vi "OwnFile20261012_Native_GetWireBroken.vi"() -> ()   [LabVIEW 2024]
panel:
  out "error out":errorcluster caption="错误输出"
  out "is_broken":bool
  in  "wire_id":u32
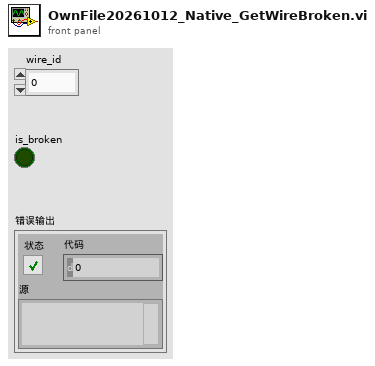
[diagram p1: front panel]
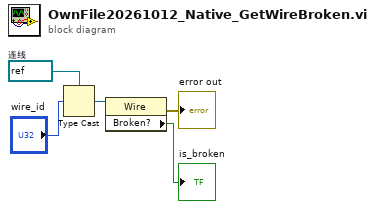
[diagram p0: block diagram]
diagram:
  w4 = refnum<vi> refnum  # 连线
  n1 = Type Cast ("强制类型转换")(type=w4, x="wire_id") -> (*(type *) &x=w3:refnum<vi>)
  n2 = property on="属性节点" class="Wire"(reference=w3) -> (error out=→"error out":errorcluster, "Broken?"=→"is_broken":bool)  [unwired: 1 in, 1 out]
